vi "Set Format and Units.vi"(8 "error in (no error)":errorcluster, 10 "Display State In":T1={"Show Axes"=FALSE, "Show Y=0"=FALSE, "Controls"={"Type"=enum."Sine", "Periods"=0.0, "Points"=0, "Offset"=0.0, "Amplitdue"=0.0, "Phase"=0.0, "func"=""}, "Show Current Location"=FALSE, "Current Location"=0, "dt"=0.0, "t0"=timestamp(0 s since 1904-01-01), "Format and Units"="%_3p"} caption="State", 11 "Cluster Control":refnum<vi>) -> (0 "error out":errorcluster, 2 "Display State Out":T1={"Show Axes"=FALSE, "Show Y=0"=FALSE, "Controls"={"Type"=enum."Sine", "Periods"=0.0, "Points"=0, "Offset"=0.0, "Amplitdue"=0.0, "Phase"=0.0, "func"=""}, "Show Current Location"=FALSE, "Current Location"=0, "dt"=0.0, "t0"=timestamp(0 s since 1904-01-01), "Format and Units"="%_3p"} caption="State")   [LabVIEW 2012, in "Waveform Control.xctl"]
doc: "Set the format and units of the Amplitude and Offset controls from the display state"
uses:
  Waveform Control.xctl
  Controls/Waveform State.ctl
  FP Controls.ctl
  Function Types.ctl
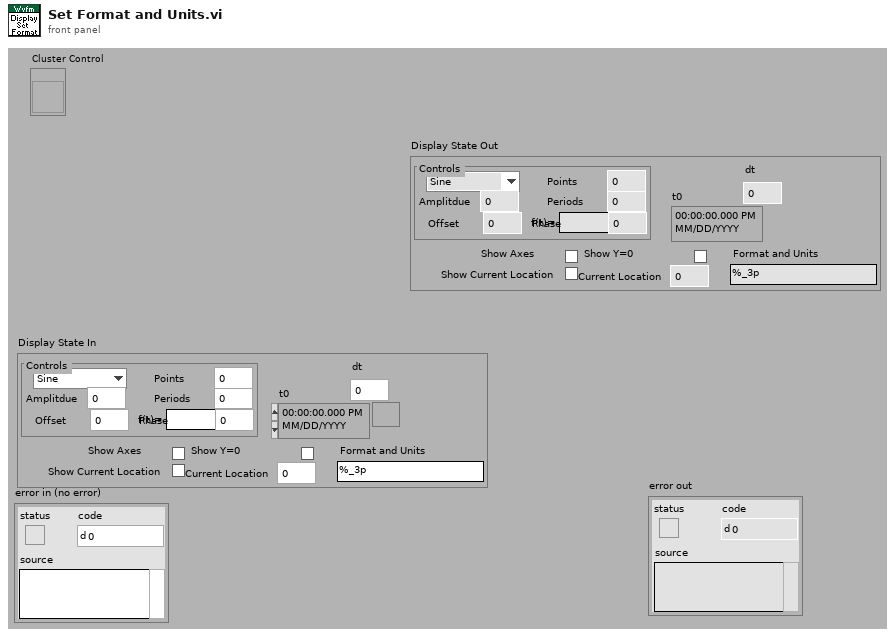
[diagram p1: front panel]
types:
  T1 = typedef "Waveform Control.xctl/Waveform State.ctl" = cluster{"Show Axes":bool, "Show Y=0":bool, "Controls":T2, "Show Current Location":bool, "Current Location":i32, "dt":dbl, "t0":timestamp, "Format and Units":string}
  T2 = typedef "Waveform Control.xctl/FP Controls.ctl" = cluster{"Type":T3, "Periods":dbl, "Points":i32, "Offset":dbl, "Amplitdue":dbl, "Phase":dbl, "func":string}
  T3 = typedef "Waveform Control.xctl/Function Types.ctl" = enum16{"Level", "Sine", "Triangle", "Ramp", "Saw Tooth", "Square", "Function"}
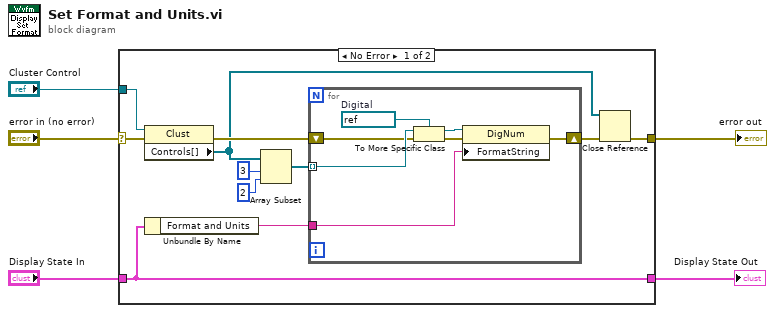
[diagram p0: block diagram]
diagram:
  n1 = case shown="No Error" "error in (no error)" {
    selector: "error in (no error)" -> [w15 w24]
    tunnel: "Display State In" -> [w6 w25]
    tunnel: "Cluster Control" -> [w16 _]
    tunnel: [w7 w24] -> w2
    tunnel: [w6 w25] -> w1
    frame No Error {
      n2 = property class="Clust"(reference=w16, error in=w15) -> (error out=w11:errorcluster, "Controls[]"=w8:refnum<vi>[])  [unwired: 1 out]
      n3 = Unbundle By Name(w6) -> ("Format and Units"=w10:string)
      n4 = Array Subset(array=w8, index=3, length=2) -> (w12:refnum<vi>[])
      n5 = for {
        tunnel: w12 -> [w23] mode=indexing
        shift-right: [w20] -> w9
        shift-left: w11 -> [w22]
        tunnel: w10 -> [w17]
        w21 = refnum<vi> refnum  # Digital
        n6 = To More Specific Class(target class=w21, reference=w23, error in=w22) -> (specific class reference=w18:refnum<vi>, error out=w19:errorcluster)
        n7 = property class="DigNum"(reference=w18, error in=w19, "FormatString"=w17) -> (error out=w20:errorcluster)  [unwired: 1 out]
      }
      n8 = Close Reference(reference=w8, error in (no error)=w9) -> (error out=w7:errorcluster)
    }
    frame Error {
    }
  }
  "Display State Out" <- w1
  "error out" <- w2
